vi "output.vi"(8 "error in":errorcluster, 10 "data table in":T1, 11 "SystemLin Tag Module runtime in":refnum<class "SystemLink File runtime.lvclass">) -> (0 "error out":errorcluster, 2 "data table out":T1, 3 "SystemLin Tag Module runtime out":refnum<class "SystemLink File runtime.lvclass">)   [LabVIEW 2015, in "SystemLink File runtime.lvclass"]
doc: "Provides an interface for writing data to a module at runtime. While this interface performs no operations, a child should provide an override which may write to any open sessions, references, or interfaces."
uses:
  SystemLink File runtime.lvclass
  <vilib>/NI/Tag Bus/table/data table.ctl
  SystemLink File runtime.lvclass/SystemLink File runtime.ctl
  <vilib>/Skyline/Configuration/Configuration AMQP_class/NI Skyline Configuration AMQP.lvclass
  <vilib>/NI/Tag Bus/table/data polymorphs/read one/read Boolean.vi
  <vilib>/Skyline/File/File/Send File.vi
  <vilib>/NI/Tag Bus/table/data table.lvlib
  <vilib>/Skyline/File/File/NI Skyline File.lvclass
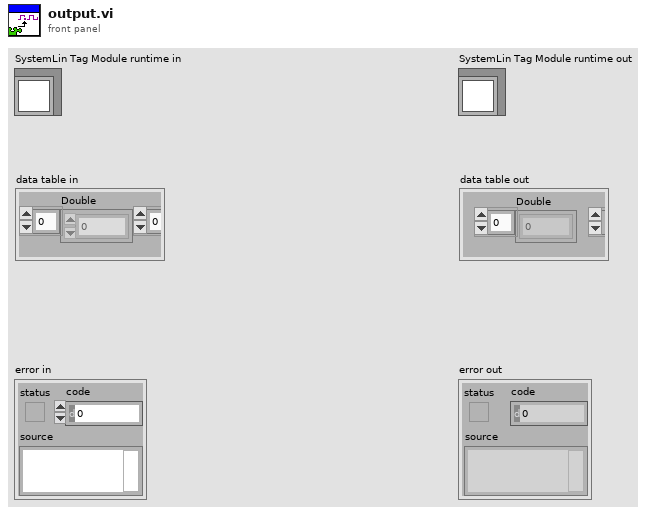
[diagram p1: front panel]
types:
  T1 = typedef "tag bus.lvlib/data table.lvlib/data table.ctl" = cluster{"Double":dbl[], "Single":sgl[], "I64":i64[], "I32":i32[], "I16":i16[], "I8":i8[], "U64":u64[], "U32":u32[], "U16":u16[], "U8":u8[], "Boolean":bool[], "String":string[], "Array of Double":cluster{"DBL Array":dbl[]}[], "Array of Single":cluster{"SGL Array":sgl[]}[], "Array of I64":cluster{"I64 Array":i64[]}[], "Array of I32":cluster{"I32 Array":i32[]}[], "Array of I16":cluster{"I16 Array":i16[]}[], "Array of I8":cluster{"I8 Array":i8[]}[], "Array of U64":cluster{"U64 Array":u64[]}[], "Array of U32":cluster{"U32 Array":u32[]}[], "Array of U16":cluster{"U16 Array":u16[]}[], "Array of U8":cluster{"U8 Array":u8[]}[], "Array of Boolean":cluster{"Boolean Array":bool[]}[], "Array of String":cluster{"String Array":string[]}[]}
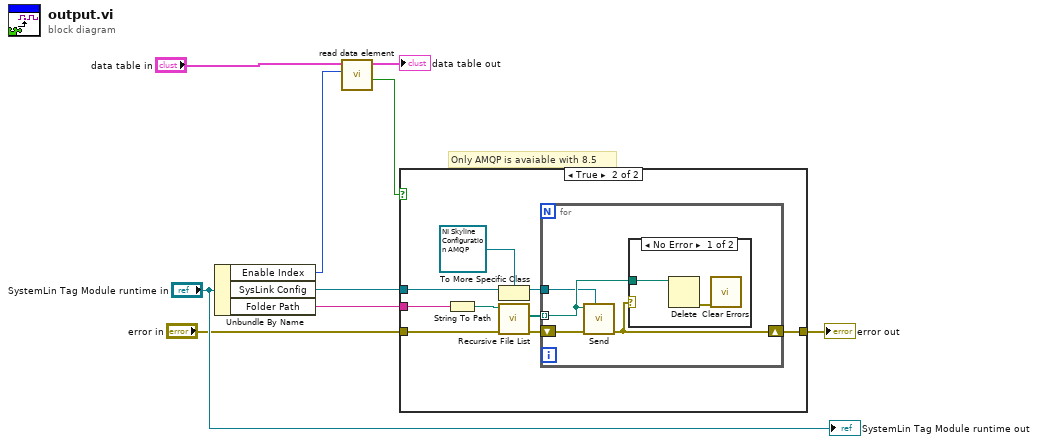
[diagram p0: block diagram]
diagram:
  # "Only AMQP is avaiable with 8.5"
  n1 = Unbundle By Name("SystemLin Tag Module runtime in") -> ("Enable Index"=w4:i32, "SysLink Config"=w2:refnum<class "NI Skyline Configuration.lvclass">, "Folder Path"=w1:string)
  n2 = call-poly <vilib>:"read data element.vi"("index"=w4, "data table in"="data table in") -> ("value"=w3:bool, "data table out"=→"data table out":T1)  [unwired: 8 in]
  n3 = case shown="True" w3 {
    tunnel: w2 -> [_ w11]
    tunnel: "error in" -> [w10 w16]
    tunnel: [w10 w19] -> w7
    tunnel: w1 -> [_ w17]
    frame False {
    }
    frame True {
      n4 = String To Path(string=w17) -> (path=w18:path)
      n5 = To More Specific Class(target class=refnum<class "NI Skyline Configuration AMQP.lvclass"> refnum ("AMQP configuration"), reference=w11) -> (specific class reference=w12:refnum<class "NI Skyline Configuration AMQP.lvclass">)  [unwired: 1 in, 1 out]
      n6 = call <vilib>:"Recursive File List.vi"("error in (no error)"=w16, "Folder Path"=w18) -> ("error out"=w15:errorcluster, "All Files in Dir"=w14:path[])  [unwired: 5 in, 3 out]
      n7 = for {
        shift-right: [w21] -> w19
        shift-left: w15 -> [w23]
        tunnel: w14 -> [w22] mode=indexing
        tunnel: w12 -> [w20]
        n8 = call-poly <vilib>:"Send.vi"("AMQP configuration"=w20, "error in (no error)"=w23, "path"=w22) -> ("error out"=w21:errorcluster)  [unwired: 6 in, 1 out]
        n9 = case shown="No Error" w21 {
          tunnel: w22 -> [w25 _]
          frame No Error {
            n10 = Delete(path (use dialog)=w25) -> (error out=w24:errorcluster)  [unwired: 4 in, 2 out]
            n11 = call <vilib>:"Clear Errors.vi"("error in (no error)"=w24) -> ()  [unwired: 5 in, 2 out]
          }
          frame Error {
          }
        }
      }
    }
  }
  "error out" <- w7
  "SystemLin Tag Module runtime out" <- "SystemLin Tag Module runtime in"
